vi "ErrBool A2.vi"(0 "flag":bool, 11 "error in":errorcluster) -> (4 "no error?":bool, 6 "error or flag?":bool)   [LabVIEW 2026]
doc: "Probe: an error cluster wired straight into Not and Or."
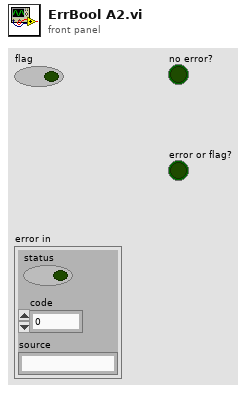
[diagram p1: front panel]
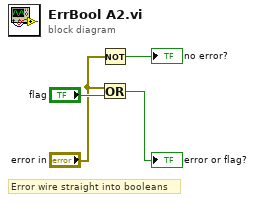
[diagram p0: block diagram]
diagram:
  # "Error wire straight into booleans"
  n1 = Not(x="error in") -> (.not. x?=→"no error?":bool)
  n2 = Or(x="error in", y="flag") -> (x .or. y?=→"error or flag?":bool)
